vi "ParseVectorFile.SVG.PathFactory.vi"(8 "error in (no error)":errorcluster, 11 "ParseVectorFile in":refnum<class "ParseVectorFile.lvclass">) -> (0 "error out":errorcluster, 3 "ParseVectorFile out":refnum<class "ParseVectorFile.lvclass">)   [LabVIEW 2019, in "ParseVectorFile.lvclass"]
uses:
  ParseVectorFile.lvclass
  ParseVectorFile.lvclass/ParseVectorFile.ctl
  ParseXML/ParseSVG.lvclass/ParseSVG.ctl
  ParsePaths/Path.lvclass
  ParseXML/ParseSVG.lvclass
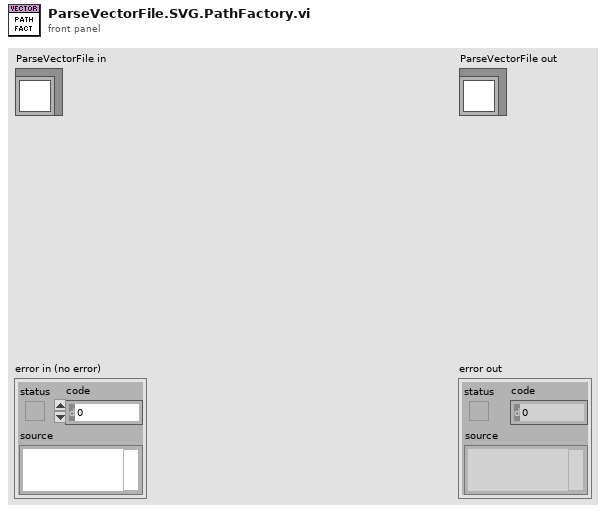
[diagram p1: front panel]
types:
  T1 = typedef "ParseSVG.lvclass/Path.ctl" = cluster{"d":string, "style":string, "transform":string, "id":string}
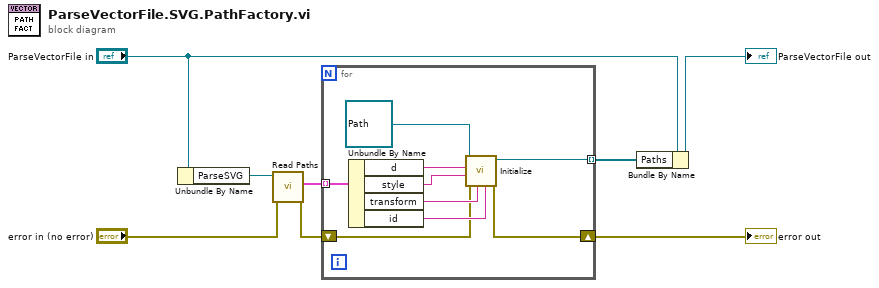
[diagram p0: block diagram]
diagram:
  n1 = Unbundle By Name("ParseVectorFile in") -> ("ParseSVG"=w8:refnum<class "ParseSVG.lvclass">)
  n2 = call "Read Paths.vi"("error in (no error)"="error in (no error)", "ParseXML in"=w8) -> ("error out"=w3:errorcluster, "Paths"=w5:T1[])  [unwired: 7 in, 1 out]
  n3 = for {
    tunnel: w5 -> [w17] mode=indexing
    shift-right: [w9] -> w2
    shift-left: w3 -> [w10]
    tunnel: [w13] -> w1 mode=indexing
    n4 = Unbundle By Name(w17) -> ("d"=w16:string, "style"=w15:string, "transform"=w11:string, "id"=w12:string)
    n5 = call "Initialize.vi"("id"=w12, "Path Transform"=w11, "error in (no error)"=w10, "Path Style"=w15, "Path Data"=w16, "Path in"=refnum<class "Path.lvclass"> refnum ("Path.lvclass")) -> ("error out"=w9:errorcluster, "Path out"=w13:refnum<class "Path.lvclass">)  [unwired: 4 in]
  }
  "error out" <- w2
  n6 = Bundle By Name(cluster="ParseVectorFile in", "Paths"=w1) -> (→"ParseVectorFile out":refnum<class "ParseVectorFile.lvclass">)
